vi "Write Query.vi"(8 "error in (no error)":errorcluster, 10 "Query":cluster{"argument":string, "value":string}[](array[cluster]), 11 "URI in":refnum<class "URI.lvclass">) -> (0 "error out":errorcluster, 3 "URI out":refnum<class "URI.lvclass">)   [LabVIEW 2013, in "openURI.lvlib" / "URI.lvclass"]
uses:
  URI.lvclass
  URI.lvclass/URI.ctl
  components/query/URI-Component.Query.lvclass
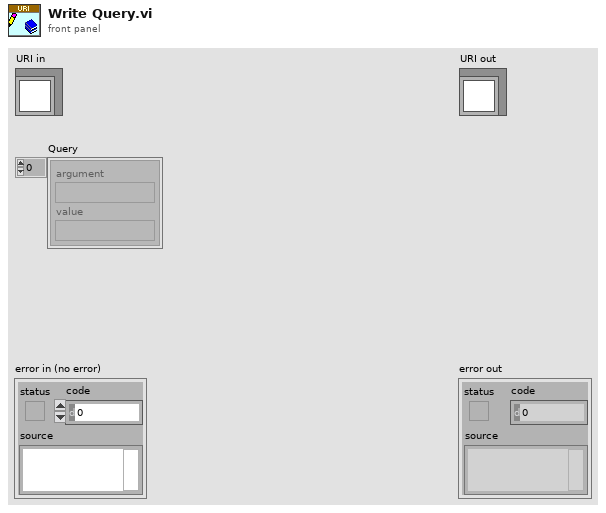
[diagram p1: front panel]
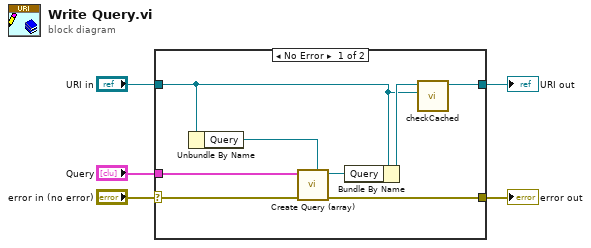
[diagram p0: block diagram]
diagram:
  n1 = case shown="No Error" "error in (no error)" {
    selector: "error in (no error)" -> [w7 w14]
    tunnel: [w6 w14] -> w4
    tunnel: [w12 w15] -> w2
    tunnel: "URI in" -> [w9 w15]
    tunnel: "Query" -> [w11 _]
    frame No Error {
      n2 = Unbundle By Name(w9) -> ("Query"=w8:refnum<class "URI-Component.Query.lvclass">)
      n3 = call "Create Query (array).vi"("URI-Component.Query"=w8, "error in (no error)"=w7, "Query"=w11) -> ("error out"=w6:errorcluster, "URI-Component.Query"=w10:refnum<class "URI-Component.Query.lvclass">)  [unwired: 7 in]
      n4 = Bundle By Name(cluster=w9, "Query"=w10) -> (w13:refnum<class "URI.lvclass">)
      n5 = call "checkCached.vi"("Old"=w9, "New URI"=w13) -> ("URI"=w12:refnum<class "URI.lvclass">)  [unwired: 9 in]
    }
    frame Error {
    }
  }
  "error out" <- w4
  "URI out" <- w2
